vi "IRregulate.vi"(8 "error in (no error)":errorcluster, 9 "Enum":T2(ring), 10 "左後距離":dbl=1.265, 11 "右後距離":dbl=1.245) -> (0 "error out":errorcluster)   [LabVIEW 2019]
uses:
  <vilib>/Platform/TimedLoop/XDataNode/timing_clust.ctl
  <vilib>/Platform/TimedLoop/XDataNode/nitl_modes.ctl
  <vilib>/Platform/TimedLoop/XDataNode/wakeup.ctl
  <vilib>/platform/TimedLoop/XDataNode/XDataNode.xnode
  <vilib>/Platform/TimedLoop/XDataNode/XDNodeRunTimeDep.lvlib
panel:
  out "Numeric":i32
  in  "左前距離":dbl=1.3
  in  "右前距離":dbl=1.3
  out "紅外線數值":T1
  out "Array":dbl[](array[numeric])
  in  "stop":bool
  out "output":dbl[](array[numeric])=[100.0, -100.0]
  out "誤差":dbl[](array[numeric])=[10401.0, -10400.0]
  in  "右邊距離":dbl
  # "4"
  # "1.28\n1.3"
  # "1.245\n1.265"
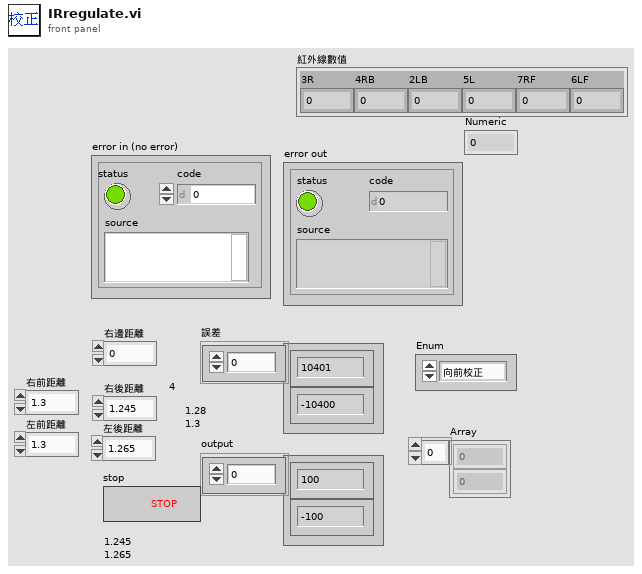
[diagram p1: front panel]
types:
  T1 = cluster{"7RF":dbl, "3R":dbl, "4RB":dbl, "5L":dbl, "6LF":dbl, "2LB":dbl}
  T2 = enum16{"向前校正", "向後校正", "右後校正", "右前校正", "左前校正", "左後校正", ""}
  T3 = typedef "AI.lvlib/AI Reference.ctl" = cluster{"myRIO Reference":T4, "AI Channels List":T8, "AI Scaling Constants List":T10}
  T4 = typedef "myRIO Generic Hardware Reference.ctl" = cluster{"myRIO Model":T5, "myRIO Hardware Reference":T6}
  T5 = typedef "Hardware Version Enum.ctl" = enum16{"Unknown", "myRIO-1900", "myRIO-1950", "roboRIO", "NI ELVIS RIO CM", "ELVIS III"}
  T6 = typedef "myRIO v1.0 Reference.ctl" = cluster{"Generic FPGA Reference":T7, "Allow multiple opens":bool}
  T7 = typedef "Generic FPGA Reference.ctl" = refnum<k20>
  T8 = typedef "AI Channels List.ctl" = T9[]
  T9 = typedef "AI Channels Enum.ctl" = enum16{"Not Connected", "AudioIn/Left", "AudioIn/Right", "C/AI0", "C/AI1", "A/AI0", "A/AI1", "A/AI2", "A/AI3", "A/AI4", "A/AI5", "A/AI6", "A/AI7", "B/AI0", "B/AI1", "B/AI2", "B/AI3", "B/AI4", "B/AI5", "B/AI6", "B/AI7", "AI/AI0", "AI/AI1", "AI/AI2", "AI/AI3", "A/AI0 (DIFF)", "A/AI1 (DIFF)", "A/AI2 (DIFF)", "A/AI3 (DIFF)", "B/AI0 (DIFF)", "B/AI1 (DIFF)", "B/AI2 (DIFF)", "B/AI3 (DIFF)"}
  T10 = typedef "Analog Scaling Constants List.ctl" = T11[]
  T11 = typedef "Analog Scaling Constants.ctl" = cluster{"LSB Weight (Volts)":dbl, "Offset (Volts)":dbl, "Signed?":bool}
  T12 = typedef "XDNodeRunTimeDep.lvlib/timing_clust.ctl" = cluster{"Expected End [f-1]":u64, "Actual End [f-1]":u64, "Finished Late? [f-1]":bool, "Expected End [i-1]":u64, "Actual End [i-1]":u64, "Finished Late? [i-1]":bool, "Expected Start [i]":u64, "Actual Start [i]":u64, "Expected Start [f]":u64, "Actual Start [f]":u64, "Source Name":string, "Structure Name":string, "Period":i64, "Deadline":i64, "Offset":i64, "Start":i64, "Priority":i32, "Timeout":i32, "Mode":T13, "Wakeup Reason":T14, "Error":errorcluster, "Source Type":string, "Secondary Source Type":string, "Global End Time":u64, "Global Start Time":u64, "Frame Duration":u64, "Iteration Duration":u64, "Assigned CPU":i32, "I/O Scan Engine Mode":u32}
  T13 = typedef "XDNodeRunTimeDep.lvlib/nitl_modes.ctl" = enum32{"No Change", "Process missed periods, maintain original phase", "Discard missed periods, maintain original phase", "Process missed periods, ignore original phase", "Discard missed periods, ignore original phase"}
  T14 = typedef "XDNodeRunTimeDep.lvlib/wakeup.ctl" = enum32{"Normal", "Aborted", "Asynchronous wakeup", "Timing source error", "Timed loop error", "Timeout"}
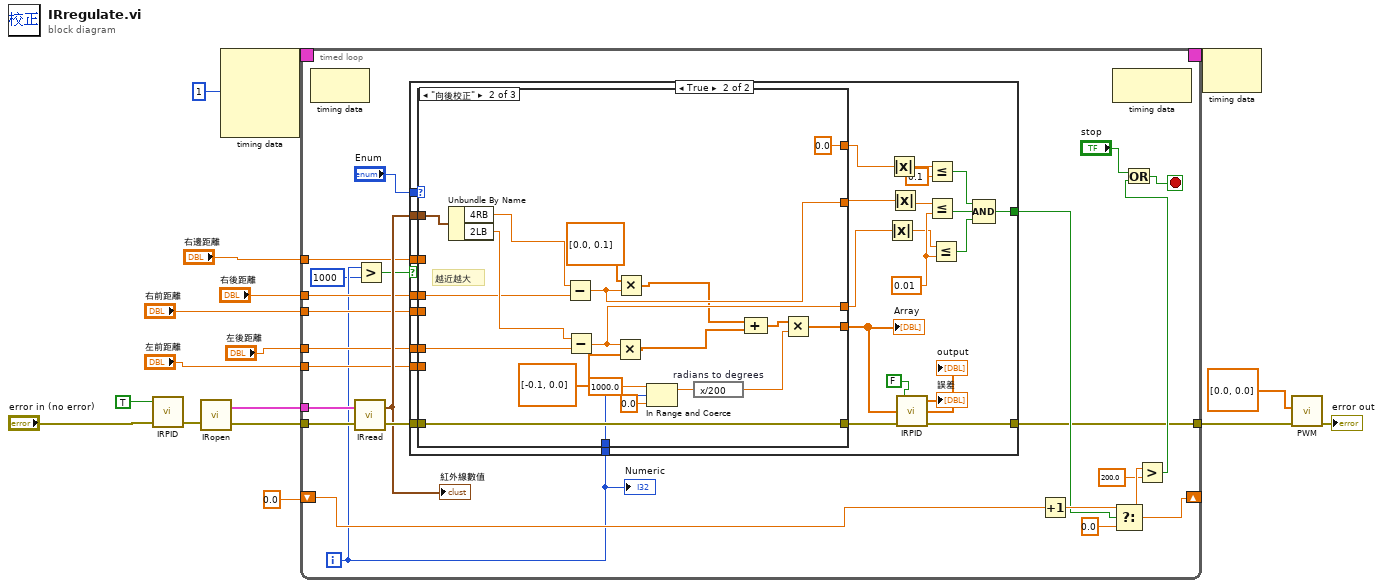
[diagram p0: block diagram]
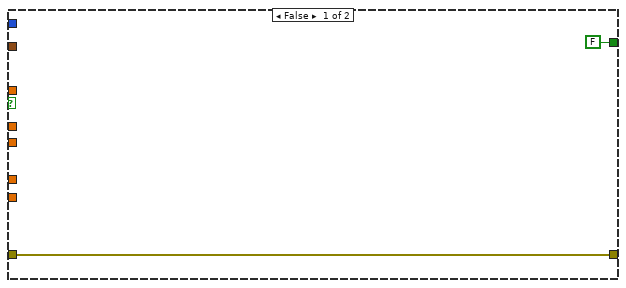
[diagram p2: hidden frame]
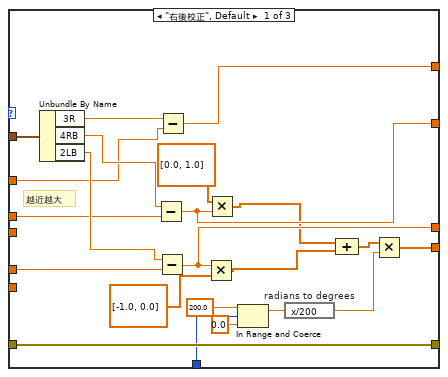
[diagram p3: hidden frame]
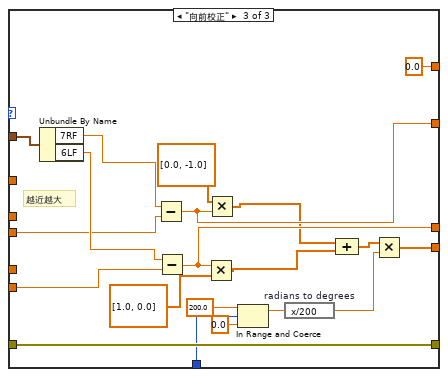
[diagram p4: hidden frame]
diagram:
  n1 = call "IRPID.vi"("error in (no error)"="error in (no error)", "Reset"=TRUE ("s")) -> ("error out"=w2:errorcluster)  [unwired: 1 in, 2 out]
  n2 = call "IRopen.vi"("error in (no error)"=w2) -> ("error out"=w15:errorcluster, "AI Ref Out"=w11:T3)  [unwired: 1 in]
  n3 = node-c288(i64 1 ("Period")) -> (w17:T12)  [unwired: 3 in]
  n4 = timed-loop {
    timing: w17 -> [_]
    timing-out: [_] -> w16
    tunnel: w15 -> [w36]
    tunnel: w11 -> [w35]
    shift-right: [w32] -> _
    shift-left: 0.0 -> [w33]
    tunnel: "右邊距離" -> [w28]
    tunnel: "右後距離" -> [w27]
    tunnel: "左後距離" -> [w26]
    tunnel: "右前距離" -> [w25]
    tunnel: "左前距離" -> [w24]
    tunnel: [w18] -> w4
    i -> [w23]
    stop <- w39 stop-if-true
    n5 = node-c288() -> ()  [unwired: 1 in, 1 out]
    n6 = call "IRread.vi"("error in (no error)"=w36, "AI Ref In"=w35) -> ("error out"=w37:errorcluster, "紅外線數值"=w29:T1)
    "紅外線數值" <- w29
    n7 = Greater?(x=w23, y=1000) -> (0:w21:bool)
    n8 = case shown="True" w21 {
      tunnel: "Enum" -> [_ w68]
      tunnel: [w42 w67] -> w18
      tunnel: w23 -> [_ w66]
      tunnel: w37 -> [w42 w65]
      tunnel: w29 -> [_ w64]
      tunnel: w28 -> [_ w63]
      tunnel: w27 -> [_ w62]
      tunnel: w26 -> [_ w61]
      tunnel: w25 -> [_ w60]
      tunnel: w24 -> [_ w59]
      tunnel: [FALSE w43] -> w19
      frame False {
      }
      frame True {
        w53 = 0.01 ("y")
        n9 = case shown="\"向後校正\"" w68 {
          tunnel: [w90 w110 w130] -> w67
          tunnel: w65 -> [w90 w110 w130]
          tunnel: [w78 w99 w119] -> w47
          tunnel: w66 -> [w83 w104 w124]
          tunnel: [w77 0.0 0.0] -> w44
          tunnel: [w76 w98 w118] -> w45
          tunnel: [w74 w96 w116] -> w46
          tunnel: w64 -> [w75 w97 w117]
          tunnel: w63 -> [w71 _ _]
          tunnel: w62 -> [w70 w93 _]
          tunnel: w61 -> [w69 w92 _]
          tunnel: w60 -> [_ _ w112]
          tunnel: w59 -> [_ _ w111]
          frame "右後校正", Default {
            # "越近越大"
            n10 = Unbundle By Name(w75) -> ("3R"=w89:dbl, "4RB"=w88:dbl, "2LB"=w87:dbl)
            n11 = Subtract(x=w88, y=w70) -> (x-y=w76:dbl)
            n12 = Subtract(x=w87, y=w69) -> (x-y=w74:dbl)
            n13 = Subtract(x=w89, y=w71) -> (x-y=w77:dbl)
            n14 = Multiply(x=w74, y=dbl[] [-1.0, 0.0] ("x")) -> (x*y=w73:dbl[])
            n15 = Multiply(x=dbl[] [0.0, 1.0], y=w76) -> (x*y=w72:dbl[])
            n16 = In Range and Coerce(upper limit=200.0, x=w83, lower limit=0.0) -> (coerced(x)=w80:dbl)  [unwired: 1 out]
            n17 = expression code="x/200" "radians to degrees"(w80) -> (w79:dbl)
            n18 = Compound Arithmetic op=ADD(w72, w73) -> (w84:dbl[])
            n19 = Multiply(x=w84, y=w79) -> (x*y=w78:dbl[])
          }
          frame "向後校正" {
            # "越近越大"
            n20 = Unbundle By Name(w97) -> ("4RB"=w109:dbl, "2LB"=w108:dbl)
            n21 = Subtract(x=w109, y=w93) -> (x-y=w98:dbl)
            n22 = Subtract(x=w108, y=w92) -> (x-y=w96:dbl)
            n23 = Multiply(x=w96, y=dbl[] [-0.1, 0.0] ("x")) -> (x*y=w95:dbl[])
            n24 = Multiply(x=dbl[] [0.0, 0.1], y=w98) -> (x*y=w94:dbl[])
            n25 = In Range and Coerce(upper limit=1000.0, x=w104, lower limit=0.0) -> (coerced(x)=w101:dbl)  [unwired: 1 out]
            n26 = expression code="x/200" "radians to degrees"(w101) -> (w100:dbl)
            n27 = Compound Arithmetic op=ADD(w94, w95) -> (w105:dbl[])
            n28 = Multiply(x=w105, y=w100) -> (x*y=w99:dbl[])
          }
          frame "向前校正" {
            # "越近越大"
            n29 = Unbundle By Name(w117) -> ("7RF"=w129:dbl, "6LF"=w128:dbl)
            n30 = Subtract(x=w129, y=w112) -> (x-y=w118:dbl)
            n31 = Subtract(x=w128, y=w111) -> (x-y=w116:dbl)
            n32 = Multiply(x=w116, y=dbl[] [1.0, 0.0] ("x")) -> (x*y=w115:dbl[])
            n33 = Multiply(x=dbl[] [0.0, -1.0], y=w118) -> (x*y=w114:dbl[])
            n34 = In Range and Coerce(upper limit=200.0, x=w124, lower limit=0.0) -> (coerced(x)=w121:dbl)  [unwired: 1 out]
            n35 = expression code="x/200" "radians to degrees"(w121) -> (w120:dbl)
            n36 = Compound Arithmetic op=ADD(w114, w115) -> (w125:dbl[])
            n37 = Multiply(x=w125, y=w120) -> (x*y=w119:dbl[])
          }
        }
        "Array" <- w47
        n38 = Absolute Value(x=w46) -> (abs(x)=w51:dbl)
        n39 = Absolute Value(x=w44) -> (abs(x)=w50:dbl)
        n40 = Absolute Value(x=w45) -> (abs(x)=w52:dbl)
        n41 = call "IRPID.vi"("目標"=w47, "Reset"=FALSE) -> ("output"=→"output":dbl[], "誤差"=→"誤差":dbl[])  [unwired: 1 in, 1 out]
        n42 = Less Or Equal?(x=w50, y=0.1) -> (x <= y?=w54:bool)
        n43 = Less Or Equal?(x=w52, y=w53) -> (x <= y?=w55:bool)
        n44 = Less Or Equal?(x=w51, y=w53) -> (x <= y?=w56:bool)
        n45 = Compound Arithmetic op=AND(w54, w55, w56) -> (w43:bool)
      }
    }
    n46 = Increment(x=w33) -> (x+1=w34:dbl)
    n47 = node-c288() -> ()  [unwired: 1 in, 1 out]
    n48 = Select(t=w34, s=w19, f=0.0) -> (s? t:f=w32:dbl)
    n49 = Greater?(x=w32, y=200.0) -> (0:w30:bool)
    n50 = Or(x="stop", y=w30) -> (x .or. y?=w39:bool)
    "Numeric" <- w23
  }
  n51 = node-c288(w16) -> ()  [unwired: 1 out]
  n52 = call "PWM.vi"("error in (no error)"=w4, "power"=dbl[] [0.0, 0.0]) -> ("error out"=→"error out":errorcluster)  [unwired: 9 in]
